vi "Test Assert In Assert Wrapper.vi"(8 "error in (no error)":errorcluster) -> (0 "error out":errorcluster)   [LabVIEW 2020]
uses:
  classes/Test/Test.lvclass
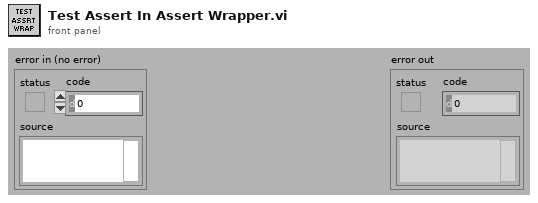
[diagram p1: front panel]
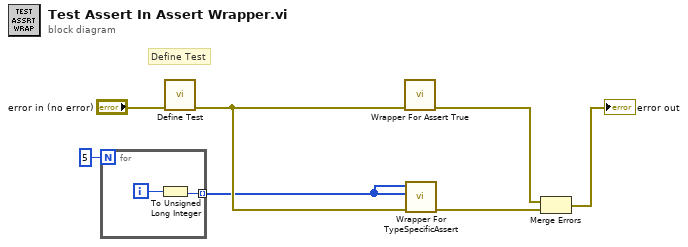
[diagram p0: block diagram]
diagram:
  # "Define Test"
  n1 = for {
    N: 5 -> [_]
    tunnel: [w8] -> w1 mode=indexing
    i -> [w9]
    n2 = To Unsigned Long Integer(number=w9) -> (unsigned 32bit integer=w8:u32)
  }
  n3 = call "Define Test.vi"("error in (no error)"="error in (no error)") -> ("error out"=w6:errorcluster)  [unwired: 9 in, 1 out]
  n4 = call "Wrapper For Assert True.vi"("error in (no error)"=w6) -> ("error out"=w4:errorcluster)  [unwired: 10 in]
  n5 = call "Wrapper For TypeSpecificAssert.vi"("error in (no error)"=w6, "U32 Array2"=w1, "U32 Array1"=w1) -> ("error out"=w5:errorcluster)  [unwired: 8 in]
  n6 = Merge Errors(w4, w5) -> (→"error out":errorcluster)
